vi "pid_controller__9a86859915.vi"(0 "set point":dbl, 1 "process variable":dbl, 3 "Output current limit":dbl(slide)=0.49999999999999994 scale=0.0..1.0, 5 "Propotional":dbl(slide) scale=0.0..1.0, 9 "Integral":dbl(slide) scale=0.0..0.01, 12 "reinitialize? (F)":bool, 13 "Derivative":dbl(slide) scale=0.0..0.01, 14 "PID dt (s)":dbl=0.003 format="%.3f") -> (4 "output":dbl, 6 "PID called time (s)":dbl format="%.3f")   [LabVIEW 2023]
uses:
  <vilib>/addons/control/pid/pid.llb/PID Control Input Filter (DBL).vi
  <vilib>/addons/control/pid/pid.llb/PID Advanced (DBL).vi
  <vilib>/addons/control/pid/NI_PID_pid.lvlib
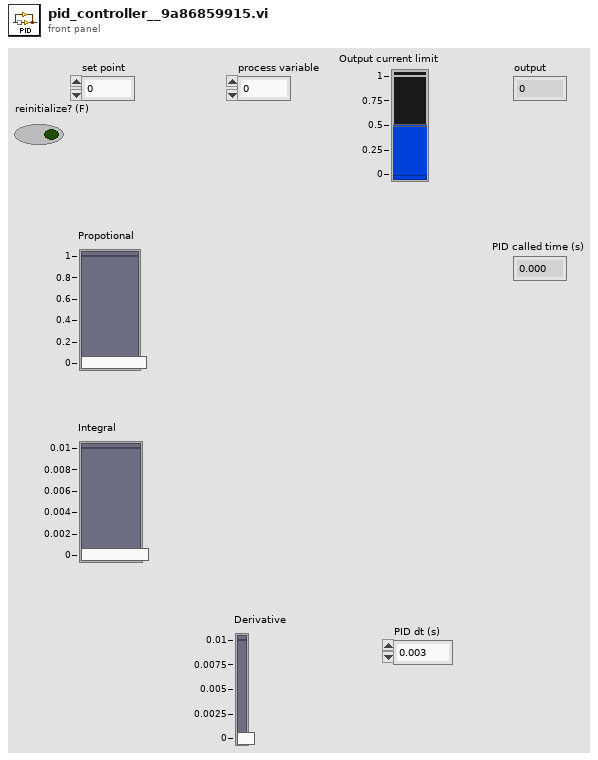
[diagram p1: front panel]
types:
  T1 = cluster{"Propotional":dbl, "Integral":dbl, "Derivative":dbl}
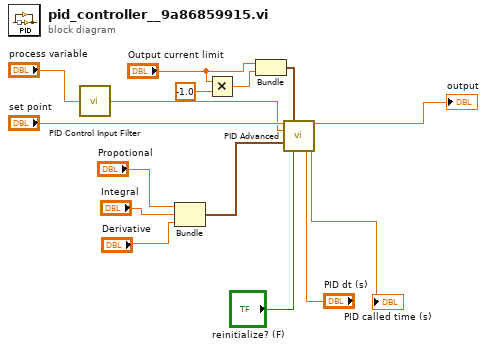
[diagram p0: block diagram]
diagram:
  n1 = call-poly <vilib>:"PID Control Input Filter.vi"("input"="process variable") -> ("output"=w13:dbl)  [unwired: 4 in]
  n2 = Bundle("Propotional"="Propotional", "Integral"="Integral", "Derivative"="Derivative") -> (w8:T1)  [unwired: 1 in]
  n3 = Multiply(x="Output current limit", y=-1.0) -> (x*y=w6:dbl)
  n4 = Bundle("Output current limit"="Output current limit", w6) -> (w7:cluster{"Output current limit ":dbl, dbl})  [unwired: 1 in]
  n5 = call-poly <vilib>:"PID Advanced.vi"("setpoint"="set point", "output range"=w7, "process variable"=w13, "PID gains"=w8, "dt (s)"="PID dt (s)", "reinitialize? (F)"="reinitialize? (F)") -> ("output"=→"output":dbl, "dt out (s)"=→"PID called time (s)":dbl)  [unwired: 8 in]
